vi "Async Core.vi"(10 "Startup Promise":refnum<class "Promise.lvclass">, 11 "Module in":refnum<class "Module.lvclass">) -> ()   [LabVIEW 2020, in "Volatus.lvlib" / "Module.lvclass"]
uses:
  Module.lvclass
  Module.lvclass/Module.ctl
  lv-promises/Promises/Promise/Promise.lvclass
  State.ctl
  MessageQ/MessageQ.lvclass
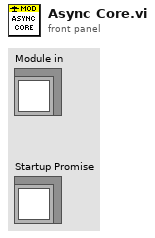
[diagram p1: front panel]
types:
  T1 = typedef "Volatus.lvlib/Module.lvclass/State.ctl" = enum16{"Unknown", "Launched", "Starting", "Running", "Stopping", "Stopped", "Error - Starting", "Error - Run", "Error - Stopping"}
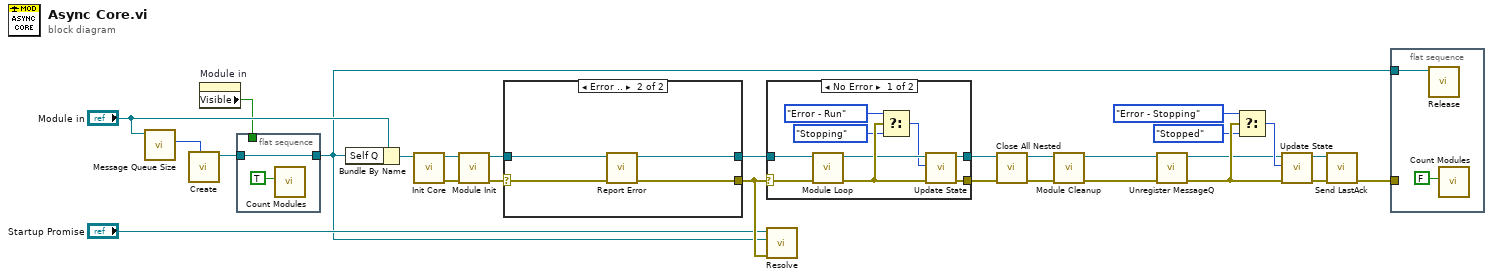
[diagram p0: block diagram]
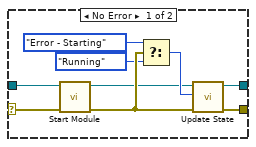
[diagram p2: hidden frame]
diagram:
  n1 = call-dynamic "Message Queue Size.vi"("Module in"="Module in") -> ("Queue Size (-1, Unlimited)"=w24:i32)  [unwired: 10 in]
  n2 = call "Create.vi"("Size (-1, Unlimited)"=w24) -> ("MessageQ out"=w25:refnum<class "MessageQ.lvclass">)  [unwired: 9 in, 1 out]
  n3 = property on="Module in" class="LVClassControl (strict)"() -> ("Visible"=w9:bool)  [unwired: 2 in, 2 out]
  n4 = flat-sequence {
    tunnel: w25 -> [w28]
    tunnel: [w28] -> w1
    tunnel: w9 -> [_]
    frame #0 {
      n5 = call "Count Modules.vi"("Increment"=TRUE) -> ()  [unwired: 11 in]
    }
  }
  n6 = Bundle By Name(cluster="Module in", "Self Q"=w1) -> (w13:refnum<class "Module.lvclass">)
  n7 = call "Init Core.vi"("Module in"=w13) -> ("error out"=w18:errorcluster, "Module out"=w21:refnum<class "Module.lvclass">)  [unwired: 9 in]
  n8 = call-dynamic "Module Init.vi"("error in (no error)"=w18, "Module in"=w21) -> ("error out"=w15:errorcluster, "Module out"=w16:refnum<class "Module.lvclass">)  [unwired: 8 in]
  n9 = case shown="Error .." w15 {
    selector: w15 -> [w36 w40]
    tunnel: w16 -> [w37 w42]
    tunnel: [w30 w39] -> w27
    tunnel: [w31 w41] -> w14
    frame No Error {
      n10 = call "Start Module.vi"("error in (no error)"=w36, "Module in"=w37) -> ("error out"=w38:errorcluster, "Module out"=w32:refnum<class "Module.lvclass">)  [unwired: 8 in]
      n11 = Select(t=State."Error - Starting" ("f"), s=w38, f=State."Running") -> (s? t:f=w33:T1)
      n12 = call "Update State.vi"("error in (no error)"=w38, "State"=w33, "Module in"=w32) -> ("error out"=w30:errorcluster, "Module out"=w31:refnum<class "Module.lvclass">)  [unwired: 7 in]
    }
    frame Error {
      n13 = call "Report Error.vi"("error in (no error)"=w40, "Module in"=w42) -> ("error out"=w39:errorcluster, "Module out"=w41:refnum<class "Module.lvclass">)  [unwired: 8 in]
    }
  }
  n14 = case shown="No Error" w27 {
    selector: w27 -> [w43 w52]
    tunnel: w14 -> [w44 w53]
    tunnel: [w48 w53] -> w11
    tunnel: [w50 w52] -> w22
    frame No Error {
      n15 = call-dynamic "Module Loop.vi"("error in (no error)"=w43, "Module in"=w44) -> ("error out"=w51:errorcluster, "Module out"=w49:refnum<class "Module.lvclass">)  [unwired: 8 in]
      n16 = Select(t=State."Error - Run" ("State"), s=w51, f=State."Stopping") -> (s? t:f=w45:T1)
      n17 = call "Update State.vi"("error in (no error)"=w51, "State"=w45, "Module in"=w49) -> ("error out"=w50:errorcluster, "Module out"=w48:refnum<class "Module.lvclass">)  [unwired: 7 in]
    }
    frame Error {
    }
  }
  n18 = call "Resolve.vi"("error in (no error)"=w27, "Result (None)"=w1, "Promise in"="Startup Promise") -> ()  [unwired: 7 in, 2 out]
  n19 = call "Close All Nested.vi"("error in (no error)"=w22, "Module in"=w11) -> ("error out"=w12:errorcluster, "Module out"=w10:refnum<class "Module.lvclass">)  [unwired: 8 in]
  n20 = call-dynamic "Module Cleanup.vi"("error in (no error)"=w12, "Module in"=w10) -> ("error out"=w26:errorcluster, "Module out"=w19:refnum<class "Module.lvclass">)  [unwired: 8 in]
  n21 = call "Unregister MessageQ.vi"("error in (no error)"=w26, "Module in"=w19) -> ("error out"=w8:errorcluster, "Module out"=w2:refnum<class "Module.lvclass">)  [unwired: 8 in]
  n22 = Select(t=State."Error - Stopping" ("State"), s=w8, f=State."Stopped") -> (s? t:f=w7:T1)
  n23 = call "Update State.vi"("error in (no error)"=w8, "State"=w7, "Module in"=w2) -> ("error out"=w4:errorcluster, "Module out"=w3:refnum<class "Module.lvclass">)  [unwired: 7 in]
  n24 = call "Send LastAck.vi"("error in (no error)"=w4, "Module in"=w3) -> ("error out"=w20:errorcluster)  [unwired: 9 in]
  n25 = flat-sequence {
    tunnel: w1 -> [w54]
    tunnel: w20 -> [_]
    frame #0 {
      n26 = call "Release.vi"("MessageQ in"=w54) -> ()  [unwired: 10 in, 1 out]
      n27 = call "Count Modules.vi"("Increment"=FALSE) -> ()  [unwired: 11 in]
    }
  }
